vi "PicoScope5000aStartStreaming.vi"(0 "error in":errorcluster, 1 "Device Info":T1, 2 "handle in":i16, 3 "Acquisition Settings":T2={"Auto Stop"=FALSE, "Desired Sample Interval"=1000, "Pre-trigger Samples"=0, "Post-trigger Samples"=1000, "Down-Sample Ratio"=1, "Down-Sample Mode"=0, "Overview Buffer Size"=15000, "Time Units"=0} {"Time Units" items=["Nanoseconds (ns)"=2, "Microseconds (us)"=3, "Milliseconds (ms)"=4, "Seconds (s)"=5]; "Down-Sample Mode" items=["None"=0, "Aggregate"=1, "Decimate"=2, "Average"=4]}, 5 "enabled array":i16[](array[numeric])) -> (6 "Channel A Buffer":i16[](array[numeric]), 7 "Port 0 Buffer":i16[](array[numeric]), 8 "Channel B Buffer":i16[](array[numeric]), 9 "Port 1 Buffer":i16[](array[numeric]), 10 "Channel C Buffer":i16[](array[numeric]), 12 "Channel D Buffer":i16[](array[numeric]), 14 "error out":errorcluster, 16 "handle out":i16, 17 "Sample Interval":u32, 19 "sampleIntervalTimeUnits":u32)   [LabVIEW 2010]
doc: "This VI starts the oscilloscope streaming. It outputs arrays that will contain samples once PicoScope3000aGetStreamingValues.vi has returned."
uses:
  ps5000a.dll
  ps5000aWrap.dll
panel:
  out "Port 1 Min Buffer":i16[](array[numeric])
  out "Port 0 Min Buffer":i16[](array[numeric])
  out "Channel D Min Buffer":i16[](array[numeric])
  out "Channel C Min Buffer":i16[](array[numeric])
  out "Channel B Min Buffer":i16[](array[numeric])
  out "Channel A Min Buffer":i16[](array[numeric])
  # "Overview Buffer Size is the size of the temporary buffers used to\nstore data before returning it to the application."
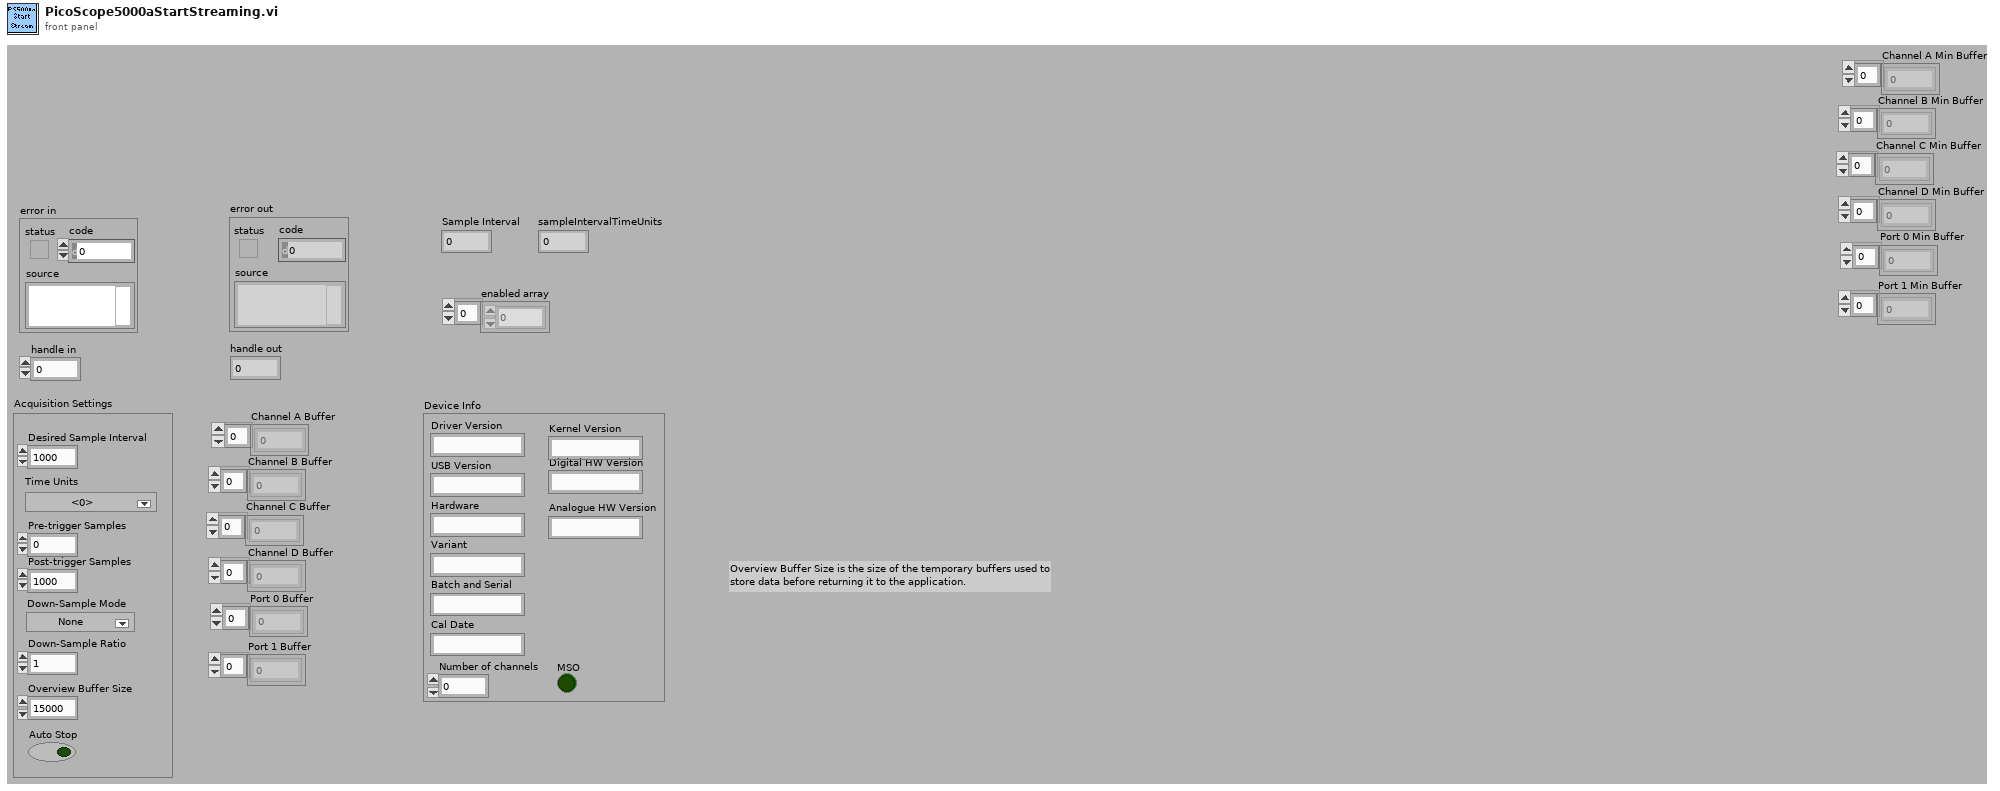
[diagram p1: front panel]
types:
  T1 = cluster{"Driver Version":string, "USB Version":string, "Hardware":string, "Variant":string, "Batch and Serial":string, "Cal Date":string, "Kernel Version":string, "Digital HW Version":string, "Analogue HW Version":string, "MSO":bool, "Number of channels":i16}
  T2 = cluster{"Auto Stop":bool, "Desired Sample Interval":u32, "Pre-trigger Samples":u32, "Post-trigger Samples":u32, "Down-Sample Ratio":u32, "Down-Sample Mode":i32, "Overview Buffer Size":u32, "Time Units":u32}
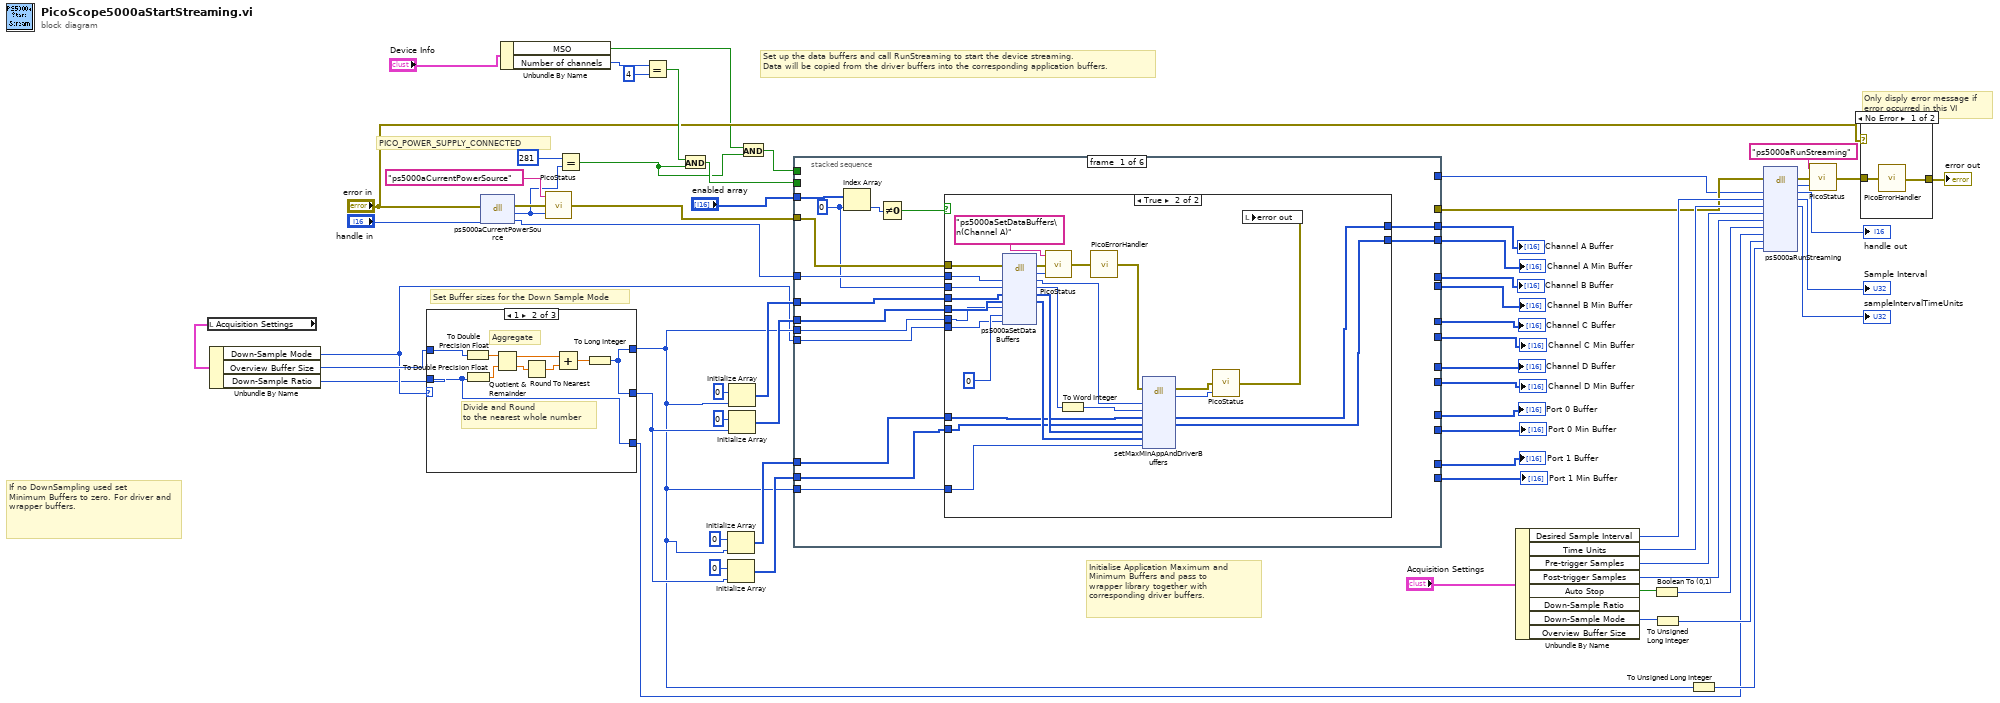
[diagram p0: block diagram]
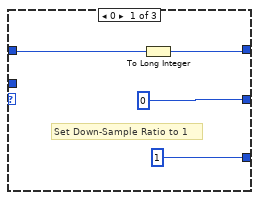
[diagram p2: hidden frame]
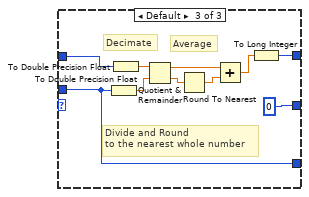
[diagram p3: hidden frame]
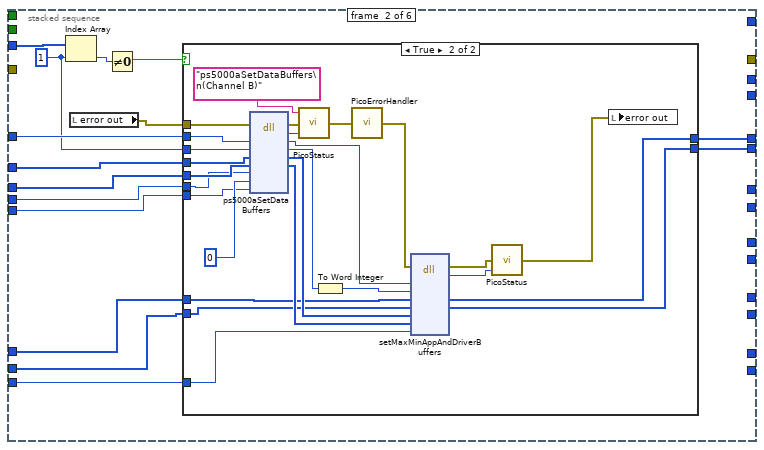
[diagram p5: hidden frame]
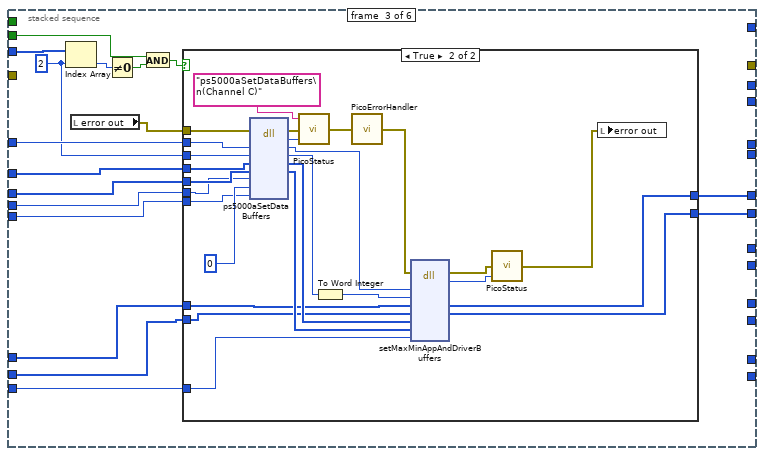
[diagram p7: hidden frame]
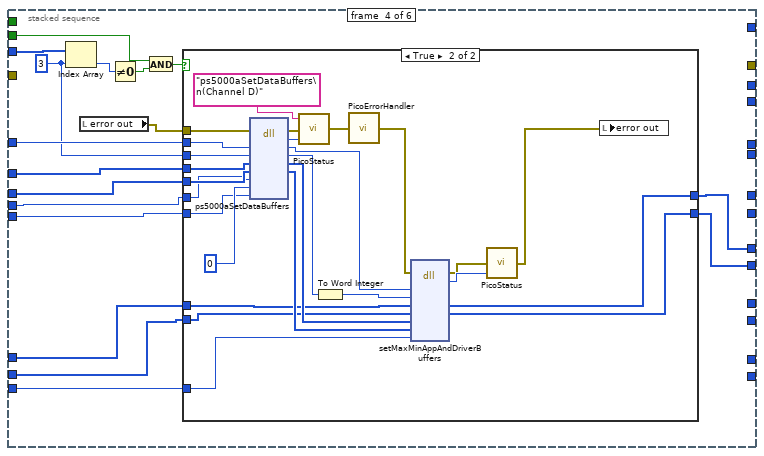
[diagram p9: hidden frame]
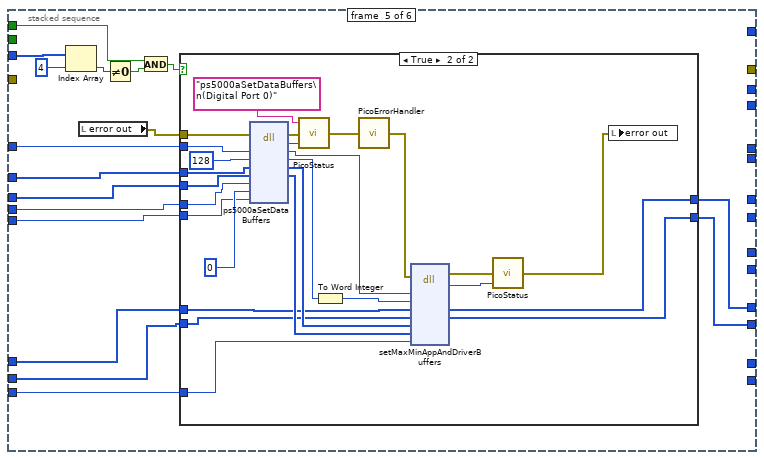
[diagram p11: hidden frame]
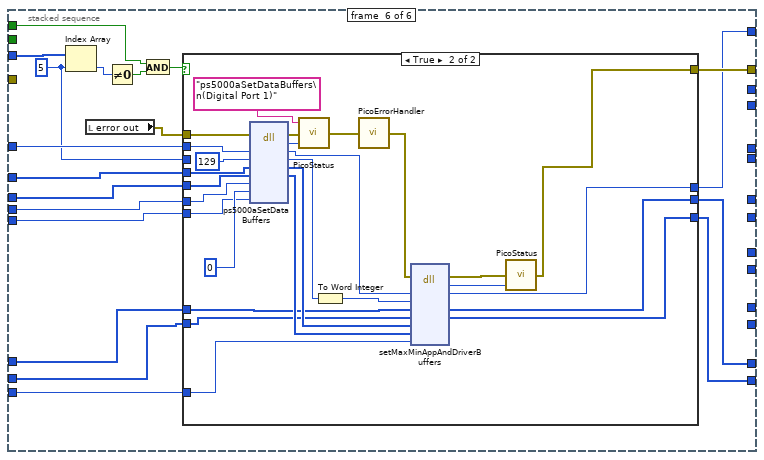
[diagram p13: hidden frame]
diagram:
  # "Set Buffer sizes for the Down Sample Mode"
  # "If no DownSampling used set \nMinimum Buffers to zero. For driver and wrapper buffers."
  # "PICO_POWER_SUPPLY_CONNECTED"
  # "Initialise Application Maximum and\nMinimum Buffers and pass to \nwrapper library together with corresponding driver buffers."
  # "Only disply error message if\nerror occurred in this VI"
  # "Set up the data buffers and call RunStreaming to start the device streaming.\nData will be copied from the driver buffers into the corresponding application buffers."
  n1 = local read "Acquisition Settings"() -> (w48:T2)
  n2 = Unbundle By Name(w48) -> ("Down-Sample Mode"=w3:i32, "Overview Buffer Size"=w4:u32, "Down-Sample Ratio"=w2:u32)
  n3 = case shown="1" w3 {
    tunnel: w2 -> [_ w69 w78]
    tunnel: w4 -> [w68 w70 w81]
    tunnel: [w67 w77 w87] -> w5
    tunnel: [0 w77 0] -> w6
    tunnel: [u32 1 ("downSampleRatio") w69 w78] -> w1
    frame 0 {
      # "Set Down-Sample Ratio to 1"
      n4 = To Long Integer(number=w68) -> (32bit integer=w67:i32)
    }
    frame 1 {
      # "Divide and Round\nto the nearest whole number"
      # "Aggregate"
      n5 = To Double Precision Float(number=w70) -> (double precision float=w73:dbl)
      n6 = To Double Precision Float(number=w69) -> (double precision float=w72:dbl)
      n7 = Quotient & Remainder(x=w73, y=w72) -> (x-y*floor(x/y)=w74:dbl, floor(x/y)=w76:dbl)
      n8 = Round To Nearest(number=w76) -> (nearest integer value=w75:dbl)
      n9 = Add(x=w74, y=w75) -> (x+y=w71:dbl)
      n10 = To Long Integer(number=w71) -> (32bit integer=w77:i32)
    }
    frame Default {
      # "Divide and Round\nto the nearest whole number"
      # "Average"
      # "Decimate"
      n11 = To Double Precision Float(number=w78) -> (double precision float=w79:dbl)
      n12 = To Double Precision Float(number=w81) -> (double precision float=w80:dbl)
      n13 = Quotient & Remainder(x=w80, y=w79) -> (x-y*floor(x/y)=w83:dbl, floor(x/y)=w85:dbl)
      n14 = Round To Nearest(number=w85) -> (nearest integer value=w84:dbl)
      n15 = Add(x=w83, y=w84) -> (x+y=w82:dbl)
      n16 = To Long Integer(number=w82) -> (32bit integer=w87:i32)
    }
  }
  n17 = dll-call lib="ps5000a.dll" fn="ps5000aCurrentPowerSource"(error in="error in", "handle"="handle in") -> (error out=w43:errorcluster, "PICO_STATUS"=w41:u32, "handle"=w33:i16)  [unwired: 2 in, 1 out]
  n18 = Unbundle By Name("Device Info") -> ("MSO"=w23:bool, "Number of channels"=w38:i16)
  n19 = call "PicoStatus.vi"("PICO STATUS"=w41, "error in"=w43, "source"="ps5000aCurrentPowerSource") -> ("error out"=w34:errorcluster)
  n20 = Equal?(x=u32 281, y=w41) -> (x = y?=w22:bool)
  n21 = Equal?(x=w38, y=i16 4) -> (x = y?=w36:bool)
  n22 = And(x=w36, y=w22) -> (x .and. y?=w26:bool)
  n23 = Initialize Array(i16 0 ("element"), w5) -> (w30:i16[])
  n24 = Initialize Array(i16 0 ("element"), w6) -> (w29:i16[])
  n25 = Initialize Array(i16 0 ("element"), w5) -> (w32:i16[])
  n26 = Initialize Array(i16 0 ("element"), w6) -> (w31:i16[])
  n27 = And(x=w23, y=w22) -> (x .and. y?=w21:bool)
  n28 = stacked-sequence {
    tunnel: "enabled array" -> [w102 w143 w186 w229 w272 w317]
    tunnel: w34 -> [w101 _ _ _ _ _]
    tunnel: w33 -> [w100 w142 w185 w228 w271 w316]
    tunnel: w32 -> [w98 w140 w183 w226 w269 w314]
    tunnel: w31 -> [w97 w139 w182 w225 w268 w313]
    tunnel: w3 -> [w96 w138 w181 w224 w267 w312]
    tunnel: w30 -> [w95 w137 w180 w223 w266 w311]
    tunnel: w29 -> [w94 w136 w179 w222 w265 w310]
    tunnel: w5 -> [w93 w135 w178 w221 w264 w309]
    tunnel: [_ _ w177 _ _ _] -> w15
    tunnel: [_ _ w176 _ _ _] -> w11
    tunnel: [_ _ _ w220 _ _] -> w16
    tunnel: [_ _ _ w219 _ _] -> w10
    tunnel: [_ _ _ _ _ w308] -> w28
    tunnel: [_ _ _ _ _ w302] -> w27
    tunnel: w26 -> [_ _ w172 w215 _ _]
    tunnel: w21 -> [_ _ _ _ w260 w304]
    tunnel: [_ _ _ _ w258 _] -> w17
    tunnel: [_ _ _ _ w257 _] -> w9
    tunnel: [_ _ _ _ _ w301] -> w18
    tunnel: [_ _ _ _ _ w300] -> w8
    tunnel: w5 -> [w91 w133 w171 w213 w256 w299]
    tunnel: [_ w132 _ _ _ _] -> w12
    tunnel: [_ w131 _ _ _ _] -> w14
    tunnel: [w90 _ _ _ _ _] -> w13
    tunnel: [w89 _ _ _ _ _] -> w19
    frame #0 {
      w99 = 0 ("index")
      n29 = Index Array(array=w102, index=w99) -> (element=w92:i16)
      n30 = Not Equal To 0?(x=w92) -> (x != 0?=w88:bool)
      n31 = case shown="True" w88 {
        tunnel: w100 -> [_ w128]
        tunnel: w101 -> [_ w127]
        tunnel: w99 -> [_ w110]
        tunnel: w98 -> [_ w117]
        tunnel: w97 -> [_ w116]
        tunnel: w96 -> [_ w115]
        tunnel: w95 -> [_ w114]
        tunnel: w94 -> [_ w113]
        tunnel: w93 -> [_ w112]
        tunnel: w91 -> [_ w105]
        tunnel: [_ w104] -> w90
        tunnel: [_ w103] -> w89
        frame False {
        }
        frame True {
          n32 = dll-call lib="ps5000a.dll" fn="ps5000aSetDataBuffers" ("ps3000.dll:_ps3000_open_unit@0")(error in=w127, "handle"=w128, "channel"=w110, "bufferMax"=w117, "bufferMin"=w116, "bufferLth"=w105, "segmentIndex"=u32 0, "downSampleRatioMode"=w115) -> (error out=w125:errorcluster, "PICO_STATUS"=w126:u32, "handle"=w122:i16, "channel"=w118:u32, "bufferMax"=w121:i16[], "bufferMin"=w120:i16[])  [unwired: 5 in, 1 out]
          n33 = call "PicoStatus.vi"("PICO STATUS"=w126, "error in"=w125, "source"="ps5000aSetDataBuffers\n(Channel A)") -> ("error out"=w111:errorcluster)
          n34 = To Word Integer(number=w118) -> (16bit integer=w119:i16)
          n35 = call "PicoErrorHandler.vi"("error in"=w111) -> ("error out"=w107:errorcluster)
          n36 = dll-call lib="ps5000aWrap.dll" fn="setMaxMinAppAndDriverBuffers" label="setMaxMinAppAndDriverBuffers \n(Channel A)"(error in=w107, "handle"=w122, "channel"=w119, "appMaxBuffer"=w114, "appMinBuffer"=w113, "driverMaxBuffer"=w121, "driverMinBuffer"=w120, "bufferLength"=w112) -> (error out=w108:errorcluster, "status"=w106:i16, "appMaxBuffer"=w103:i16[], "appMinBuffer"=w104:i16[])  [unwired: 7 in, 1 out]
          n37 = call "PicoStatus.vi"("PICO STATUS"=w106, "error in"=w108) -> ("error out"=w109:errorcluster)  [unwired: 1 in]
          n38 = local write "error out"(w109) -> ()
        }
      }
    }
    frame #1 {
      w141 = 1 ("index")
      n39 = Index Array(array=w143, index=w141) -> (element=w134:i16)
      n40 = local read "error out"() -> (w130:errorcluster)
      n41 = Not Equal To 0?(x=w134) -> (x != 0?=w129:bool)
      n42 = case shown="True" w129 {
        tunnel: w142 -> [_ w169]
        tunnel: w130 -> [_ w168]
        tunnel: w141 -> [_ w151]
        tunnel: w140 -> [_ w158]
        tunnel: w139 -> [_ w157]
        tunnel: w138 -> [_ w156]
        tunnel: w137 -> [_ w155]
        tunnel: w136 -> [_ w154]
        tunnel: w135 -> [_ w153]
        tunnel: w133 -> [_ w146]
        tunnel: [_ w145] -> w132
        tunnel: [_ w144] -> w131
        frame False {
        }
        frame True {
          n43 = dll-call lib="ps5000a.dll" fn="ps5000aSetDataBuffers" ("ps3000.dll:_ps3000_open_unit@0")(error in=w168, "handle"=w169, "channel"=w151, "bufferMax"=w158, "bufferMin"=w157, "bufferLth"=w146, "segmentIndex"=u32 0, "downSampleRatioMode"=w156) -> (error out=w166:errorcluster, "PICO_STATUS"=w167:u32, "handle"=w163:i16, "channel"=w159:u32, "bufferMax"=w162:i16[], "bufferMin"=w161:i16[])  [unwired: 5 in, 1 out]
          n44 = call "PicoStatus.vi"("PICO STATUS"=w167, "error in"=w166, "source"="ps5000aSetDataBuffers\n(Channel B)") -> ("error out"=w152:errorcluster)
          n45 = To Word Integer(number=w159) -> (16bit integer=w160:i16)
          n46 = call "PicoErrorHandler.vi"("error in"=w152) -> ("error out"=w148:errorcluster)
          n47 = dll-call lib="ps5000aWrap.dll" fn="setMaxMinAppAndDriverBuffers" label="setMaxMinAppAndDriverBuffers \n(Channel B)"(error in=w148, "handle"=w163, "channel"=w160, "appMaxBuffer"=w155, "appMinBuffer"=w154, "driverMaxBuffer"=w162, "driverMinBuffer"=w161, "bufferLength"=w153) -> (error out=w149:errorcluster, "status"=w147:i16, "appMaxBuffer"=w144:i16[], "appMinBuffer"=w145:i16[])  [unwired: 7 in, 1 out]
          n48 = call "PicoStatus.vi"("PICO STATUS"=w147, "error in"=w149) -> ("error out"=w150:errorcluster)  [unwired: 1 in]
          n49 = local write "error out"(w150) -> ()
        }
      }
    }
    frame #2 {
      w184 = 2 ("index")
      n50 = Index Array(array=w186, index=w184) -> (element=w173:i16)
      n51 = local read "error out"() -> (w170:errorcluster)
      n52 = Not Equal To 0?(x=w173) -> (x != 0?=w175:bool)
      n53 = And(x=w172, y=w175) -> (x .and. y?=w174:bool)
      n54 = case shown="True" w174 {
        tunnel: w185 -> [_ w212]
        tunnel: w170 -> [_ w211]
        tunnel: w184 -> [_ w192]
        tunnel: w183 -> [_ w201]
        tunnel: w182 -> [_ w200]
        tunnel: w181 -> [_ w199]
        tunnel: w180 -> [_ w198]
        tunnel: w179 -> [_ w197]
        tunnel: w178 -> [_ w196]
        tunnel: [_ w195] -> w177
        tunnel: [_ w194] -> w176
        tunnel: w171 -> [_ w187]
        frame False {
        }
        frame True {
          n55 = dll-call lib="ps5000a.dll" fn="ps5000aSetDataBuffers" ("ps3000.dll:_ps3000_open_unit@0")(error in=w211, "handle"=w212, "channel"=w192, "bufferMax"=w201, "bufferMin"=w200, "bufferLth"=w187, "segmentIndex"=u32 0, "downSampleRatioMode"=w199) -> (error out=w209:errorcluster, "PICO_STATUS"=w210:u32, "handle"=w206:i16, "channel"=w202:u32, "bufferMax"=w205:i16[], "bufferMin"=w204:i16[])  [unwired: 5 in, 1 out]
          n56 = call "PicoStatus.vi"("PICO STATUS"=w210, "error in"=w209, "source"="ps5000aSetDataBuffers\n(Channel C)") -> ("error out"=w193:errorcluster)
          n57 = To Word Integer(number=w202) -> (16bit integer=w203:i16)
          n58 = call "PicoErrorHandler.vi"("error in"=w193) -> ("error out"=w189:errorcluster)
          n59 = dll-call lib="ps5000aWrap.dll" fn="setMaxMinAppAndDriverBuffers" label="setMaxMinAppAndDriverBuffers \n(Channel C)"(error in=w189, "handle"=w206, "channel"=w203, "appMaxBuffer"=w198, "appMinBuffer"=w197, "driverMaxBuffer"=w205, "driverMinBuffer"=w204, "bufferLength"=w196) -> (error out=w190:errorcluster, "status"=w188:i16, "appMaxBuffer"=w195:i16[], "appMinBuffer"=w194:i16[])  [unwired: 7 in, 1 out]
          n60 = call "PicoStatus.vi"("PICO STATUS"=w188, "error in"=w190) -> ("error out"=w191:errorcluster)  [unwired: 1 in]
          n61 = local write "error out"(w191) -> ()
        }
      }
    }
    frame #3 {
      w227 = 3 ("index")
      n62 = Index Array(array=w229, index=w227) -> (element=w216:i16)
      n63 = local read "error out"() -> (w214:errorcluster)
      n64 = Not Equal To 0?(x=w216) -> (x != 0?=w218:bool)
      n65 = And(x=w215, y=w218) -> (x .and. y?=w217:bool)
      n66 = case shown="True" w217 {
        tunnel: w228 -> [_ w255]
        tunnel: w214 -> [_ w254]
        tunnel: w227 -> [_ w244]
        tunnel: w226 -> [_ w243]
        tunnel: w225 -> [_ w242]
        tunnel: w224 -> [_ w241]
        tunnel: w223 -> [_ w240]
        tunnel: w222 -> [_ w239]
        tunnel: w221 -> [_ w238]
        tunnel: [_ w237] -> w220
        tunnel: [_ w236] -> w219
        tunnel: w213 -> [_ w230]
        frame False {
        }
        frame True {
          n67 = dll-call lib="ps5000a.dll" fn="ps5000aSetDataBuffers" ("ps3000.dll:_ps3000_open_unit@0")(error in=w254, "handle"=w255, "channel"=w244, "bufferMax"=w243, "bufferMin"=w242, "bufferLth"=w230, "segmentIndex"=u32 0, "downSampleRatioMode"=w241) -> (error out=w252:errorcluster, "PICO_STATUS"=w253:u32, "handle"=w249:i16, "channel"=w245:u32, "bufferMax"=w248:i16[], "bufferMin"=w247:i16[])  [unwired: 5 in, 1 out]
          n68 = call "PicoStatus.vi"("PICO STATUS"=w253, "error in"=w252, "source"="ps5000aSetDataBuffers\n(Channel D)") -> ("error out"=w235:errorcluster)
          n69 = To Word Integer(number=w245) -> (16bit integer=w246:i16)
          n70 = call "PicoErrorHandler.vi"("error in"=w235) -> ("error out"=w231:errorcluster)
          n71 = dll-call lib="ps5000aWrap.dll" fn="setMaxMinAppAndDriverBuffers" label="setMaxMinAppAndDriverBuffers \n(Channel D)"(error in=w231, "handle"=w249, "channel"=w246, "appMaxBuffer"=w240, "appMinBuffer"=w239, "driverMaxBuffer"=w248, "driverMinBuffer"=w247, "bufferLength"=w238) -> (error out=w233:errorcluster, "status"=w234:i16, "appMaxBuffer"=w237:i16[], "appMinBuffer"=w236:i16[])  [unwired: 7 in, 1 out]
          n72 = call "PicoStatus.vi"("PICO STATUS"=w234, "error in"=w233) -> ("error out"=w232:errorcluster)  [unwired: 1 in]
          n73 = local write "error out"(w232) -> ()
        }
      }
    }
    frame #4 {
      n74 = Index Array(array=w272, index=4) -> (element=w261:i16)
      n75 = local read "error out"() -> (w259:errorcluster)
      n76 = Not Equal To 0?(x=w261) -> (x != 0?=w262:bool)
      n77 = And(x=w260, y=w262) -> (x .and. y?=w263:bool)
      n78 = case shown="True" w263 {
        tunnel: w271 -> [_ w298]
        tunnel: w259 -> [_ w297]
        tunnel: w269 -> [_ w287]
        tunnel: w268 -> [_ w286]
        tunnel: w267 -> [_ w285]
        tunnel: w266 -> [_ w284]
        tunnel: w265 -> [_ w283]
        tunnel: w264 -> [_ w282]
        tunnel: [_ w281] -> w258
        tunnel: [_ w280] -> w257
        tunnel: w256 -> [_ w273]
        frame False {
        }
        frame True {
          n79 = dll-call lib="ps5000a.dll" fn="ps5000aSetDataBuffers" ("ps3000.dll:_ps3000_open_unit@0")(error in=w297, "handle"=w298, "channel"=u32 128, "bufferMax"=w287, "bufferMin"=w286, "bufferLth"=w273, "segmentIndex"=u32 0, "downSampleRatioMode"=w285) -> (error out=w295:errorcluster, "PICO_STATUS"=w296:u32, "handle"=w292:i16, "channel"=w288:u32, "bufferMax"=w291:i16[], "bufferMin"=w290:i16[])  [unwired: 5 in, 1 out]
          n80 = call "PicoStatus.vi"("PICO STATUS"=w296, "error in"=w295, "source"="ps5000aSetDataBuffers\n(Digital Port 0)") -> ("error out"=w278:errorcluster)
          n81 = To Word Integer(number=w288) -> (16bit integer=w289:i16)
          n82 = call "PicoErrorHandler.vi"("error in"=w278) -> ("error out"=w274:errorcluster)
          n83 = dll-call lib="ps5000aWrap.dll" fn="setMaxMinAppAndDriverBuffers" label="setMaxMinAppAndDriverBuffers \n(Digital Port 0)"(error in=w274, "handle"=w292, "channel"=w289, "appMaxBuffer"=w284, "appMinBuffer"=w283, "driverMaxBuffer"=w291, "driverMinBuffer"=w290, "bufferLength"=w282) -> (error out=w276:errorcluster, "status"=w277:i16, "appMaxBuffer"=w281:i16[], "appMinBuffer"=w280:i16[])  [unwired: 7 in, 1 out]
          n84 = call "PicoStatus.vi"("PICO STATUS"=w277, "error in"=w276) -> ("error out"=w275:errorcluster)  [unwired: 1 in]
          n85 = local write "error out"(w275) -> ()
        }
      }
    }
    frame #5 {
      w315 = 5 ("index")
      n86 = Index Array(array=w317, index=w315) -> (element=w305:i16)
      n87 = local read "error out"() -> (w303:errorcluster)
      n88 = Not Equal To 0?(x=w305) -> (x != 0?=w307:bool)
      n89 = And(x=w304, y=w307) -> (x .and. y?=w306:bool)
      n90 = case shown="True" w306 {
        tunnel: w316 -> [w318 w346]
        tunnel: w303 -> [w319 w345]
        tunnel: w315 -> [_ _]
        tunnel: w314 -> [_ w335]
        tunnel: w313 -> [_ w334]
        tunnel: w312 -> [_ w333]
        tunnel: w311 -> [_ w332]
        tunnel: w310 -> [_ w331]
        tunnel: w309 -> [_ w330]
        tunnel: [_ w329] -> w301
        tunnel: [_ w328] -> w300
        tunnel: [w319 w323] -> w308
        tunnel: [w318 w327] -> w302
        tunnel: w299 -> [_ w320]
        frame False {
        }
        frame True {
          n91 = dll-call lib="ps5000a.dll" fn="ps5000aSetDataBuffers" ("ps3000.dll:_ps3000_open_unit@0")(error in=w345, "handle"=w346, "channel"=u32 129, "bufferMax"=w335, "bufferMin"=w334, "bufferLth"=w320, "segmentIndex"=u32 0, "downSampleRatioMode"=w333) -> (error out=w343:errorcluster, "PICO_STATUS"=w344:u32, "handle"=w340:i16, "channel"=w336:u32, "bufferMax"=w339:i16[], "bufferMin"=w338:i16[])  [unwired: 5 in, 1 out]
          n92 = call "PicoStatus.vi"("PICO STATUS"=w344, "error in"=w343, "source"="ps5000aSetDataBuffers\n(Digital Port 1)") -> ("error out"=w326:errorcluster)
          n93 = To Word Integer(number=w336) -> (16bit integer=w337:i16)
          n94 = call "PicoErrorHandler.vi"("error in"=w326) -> ("error out"=w322:errorcluster)
          n95 = dll-call lib="ps5000aWrap.dll" fn="setMaxMinAppAndDriverBuffers" label="setMaxMinAppAndDriverBuffers \n(Digital Port 1)"(error in=w322, "handle"=w340, "channel"=w337, "appMaxBuffer"=w332, "appMinBuffer"=w331, "driverMaxBuffer"=w339, "driverMinBuffer"=w338, "bufferLength"=w330) -> (error out=w321:errorcluster, "status"=w324:i16, "handle"=w327:i16, "appMaxBuffer"=w329:i16[], "appMinBuffer"=w328:i16[])  [unwired: 6 in, 1 out]
          n96 = call "PicoStatus.vi"("PICO STATUS"=w324, "error in"=w321) -> ("error out"=w323:errorcluster)  [unwired: 1 in]
        }
      }
    }
  }
  "Channel A Buffer" <- w19
  "Channel B Buffer" <- w14
  "Channel C Buffer" <- w15
  "Channel D Buffer" <- w16
  "Port 0 Buffer" <- w17
  "Port 1 Buffer" <- w18
  "Channel A Min Buffer" <- w13
  "Channel B Min Buffer" <- w12
  "Channel C Min Buffer" <- w11
  "Channel D Min Buffer" <- w10
  "Port 0 Min Buffer" <- w9
  "Port 1 Min Buffer" <- w8
  n97 = Unbundle By Name("Acquisition Settings") -> ("Desired Sample Interval"=w56:u32, "Time Units"=w47:u32, "Pre-trigger Samples"=w55:u32, "Post-trigger Samples"=w54:u32, "Auto Stop"=w53:bool, "Down-Sample Mode"=w49:i32)  [unwired: 2 out]
  n98 = Boolean To (0,1)(Boolean=w53) -> (0, 1=w57:i16)
  n99 = To Unsigned Long Integer(number=w49) -> (unsigned 32bit integer=w40:u32)
  n100 = To Unsigned Long Integer(number=w5) -> (unsigned 32bit integer=w7:u32)
  n101 = dll-call lib="ps5000a.dll" fn="ps5000aRunStreaming" ("ps5000a.dll:_ps3000_open_unit@0")(error in=w28, "handle"=w27, "sampleInterval"=w56, "sampleIntervalTimeUnits"=w47, "maxPreTriggerSamples"=w55, "maxPostTriggerSamples"=w54, "autoStop"=w57, "downSampleRatio"=w1, "downSampleRatioMode"=w40, "overviewBufferSize"=w7) -> (error out=w61:errorcluster, "PICO_STATUS"=w62:u32, "handle"=→"handle out":i16, "sampleInterval"=→"Sample Interval":u32, "sampleIntervalTimeUnits"=→"sampleIntervalTimeUnits":u32)  [unwired: 8 in, 1 out]
  n102 = call "PicoStatus.vi"("PICO STATUS"=w62, "error in"=w61, "source"="ps5000aRunStreaming") -> ("error out"=w59:errorcluster)
  n103 = case shown="No Error" "error in" {
    tunnel: [w348 w349] -> w64
    tunnel: w59 -> [w347 w349]
    frame No Error {
      n104 = call "PicoErrorHandler.vi"("error in"=w347) -> ("error out"=w348:errorcluster)
    }
    frame Error {
    }
  }
  "error out" <- w64
